vi "getSerializedData.vi"(0 "reference":refnum<class "NoteNode.lvclass">, 5 "error in (no error)":errorcluster) -> (14 "reference out":refnum<class "NoteNode.lvclass">, 15 "parent":refnum<class "AbstractNode.lvclass">, 16 "children":refnum<class "AbstractNode.lvclass">[](array[class]), 17 "xmlOut":string, 19 "error out":errorcluster)   [LabVIEW 2020, in "NoteNode.lvclass"]
doc: "getSerializedData"
uses:
  <resource>/Framework/Providers/Open_GDS/UML/NoteNode_class/NoteNode.lvclass
  C:/Program Files (x86)/National Instruments/LabVIEW 2020/resource/Framework/Providers/Open_GDS/UML/RectangularNode_class/RectangularNode.lvclass
  C:/Program Files (x86)/National Instruments/LabVIEW 2020/resource/Framework/Providers/Open_GDS/UML/AbstractNode_class/AbstractNode.lvclass
  <resource>/Framework/Providers/Open_GDS/UML/AbstractNode_class/AbstractNode.lvclass
  <resource>/Framework/Providers/Open_GDS/UML/General/Rectangle/Rectangle Rectangle2D.ctl
  <resource>/Framework/Providers/Open_GDS/UML/MultiLineString_class/JustificationType.ctl
  <resource>/Framework/Providers/Open_GDS/UML/MultiLineString_class/MultiLineString.lvclass
  <resource>/Framework/Providers/Open_GDS/UML/RectangularNode_class/RectangularNode.lvclass
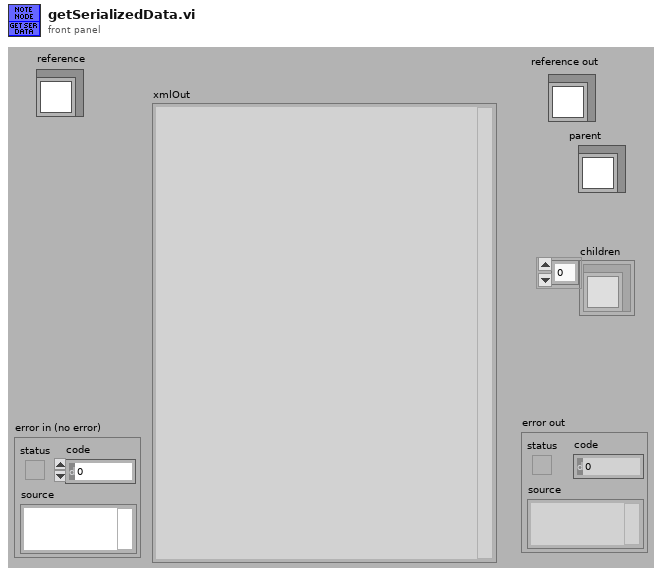
[diagram p1: front panel]
types:
  T1 = typedef "Rectangle Rectangle2D.ctl" = cluster{"x":dbl, "y":dbl, "width":dbl, "height":dbl}
  T2 = cluster{"Base class":cluster{"Base class":cluster{"parent":refnum<k1>, "children":refnum<k1>[], "Hidden":bool}, "bounds":T1}, "DEFAULT_WIDTH":i32, "DEFAULT_HEIGHT":i32, "DEFAULT_COLOR":u32, "FOLD_X":i32, "FOLD_Y":i32, "color":u32, "text":refnum<k1>, "pointNodes":refnum<k1>[]}
  T3 = typedef "MultiLineString.lvclass/JustificationType.ctl" = enum16{"LEFT", "CENTER", "RIGHT"}
  T4 = typedef "NoteNode.lvclass/ObjectAttributes.ctl" = cluster{"DEFAULT_WIDTH":i32, "DEFAULT_HEIGHT":i32, "DEFAULT_COLOR":u32, "FOLD_X":i32, "FOLD_Y":i32, "color":u32, "text":refnum<class "MultiLineString.lvclass">, "pointNodes":refnum<class "AbstractNode.lvclass">[]}
  T5 = typedef "RectangularNode.lvclass/ObjectAttributes.ctl" = cluster{"bounds":T1}
  T6 = typedef "AbstractNode.lvclass/ObjectAttributes.ctl" = cluster{"parent":refnum<class "AbstractNode.lvclass">, "children":refnum<class "AbstractNode.lvclass">[], "Hidden":bool}
  T7 = cluster{"Attributes":cluster{"Base class":cluster{"Base class":cluster{"parent":refnum<k1>, "children":refnum<k1>[], "Hidden":bool}, "bounds":T1}, "DEFAULT_WIDTH":i32, "DEFAULT_HEIGHT":i32, "DEFAULT_COLOR":u32, "FOLD_X":i32, "FOLD_Y":i32, "color":u32, "text":refnum<k1>, "pointNodes":refnum<k1>[]}, string}
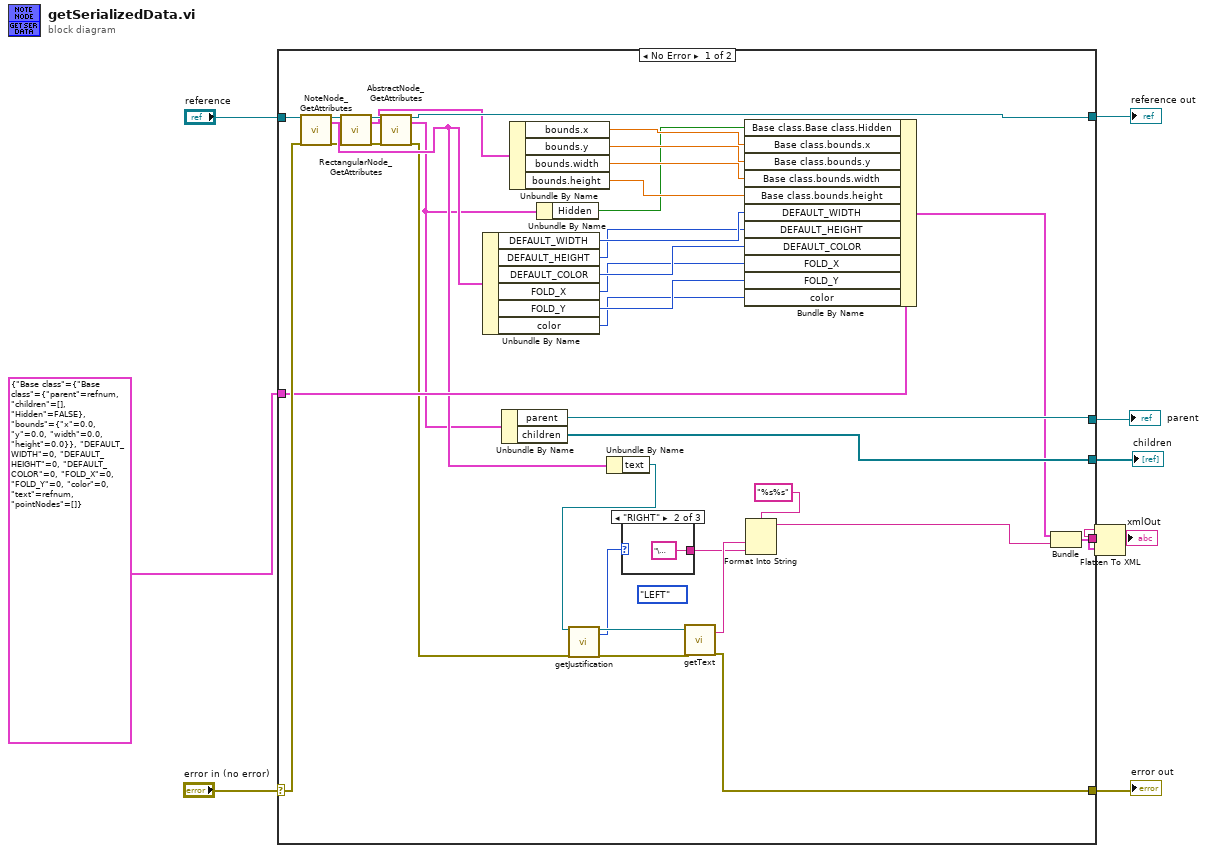
[diagram p0: block diagram]
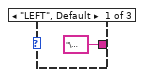
[diagram p2: hidden frame]
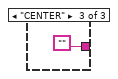
[diagram p3: hidden frame]
diagram:
  n1 = case shown="No Error" "error in (no error)" {
    selector: "error in (no error)" -> [w45 w49]
    tunnel: "reference" -> [w44 w50]
    tunnel: [w42 w49] -> w6
    tunnel: [w11 w50] -> w5
    tunnel: [w41 _] -> w4
    tunnel: [w40 _] -> w3
    tunnel: [w39 _] -> w2
    tunnel: T2 {"Base class"={"Base class"={"parent"=refnum, "children"=[], "Hidden"=FALSE}, "bounds"={"x"=0.0, "y"=0.0, "width"=0.0, "height"=0.0}}, "DEFAULT_WIDTH"=0, "DEFAULT_HEIGHT"=0, "DEFAULT_COLOR"=0, "FOLD_X"=0, "FOLD_Y"=0, "color"=0, "text"=refnum, "pointNodes"=[]} ("Attributes") -> [w30 _]
    frame No Error {
      (unwired) JustificationType."LEFT" ("justification")
      n2 = call <resource>:"NoteNode_GetAttributes.vi"("reference in"=w44, "error in (no error)"=w45) -> ("reference out"=w16:refnum<class "NoteNode.lvclass">, "Data"=w17:T4, "error out"=w15:errorcluster)  [unwired: 1 in, 14 out]
      n3 = call <resource>:"RectangularNode_GetAttributes.vi"("reference in"=w16, "error in (no error)"=w15) -> ("reference out"=w14:refnum<class "NoteNode.lvclass">, "Data"=w9:T5, "error out"=w13:errorcluster)  [unwired: 14 in, 1 out]
      n4 = call <resource>:"AbstractNode_GetAttributes.vi"("reference in"=w14, "error in (no error)"=w13) -> ("reference out"=w11:refnum<class "NoteNode.lvclass">, "Data"=w10:T6, "error out"=w12:errorcluster)  [unwired: 14 in, 1 out]
      n5 = Unbundle By Name(w17) -> ("DEFAULT_WIDTH"=w25:i32, "DEFAULT_HEIGHT"=w24:i32, "DEFAULT_COLOR"=w23:u32, "FOLD_X"=w22:i32, "FOLD_Y"=w21:i32, "color"=w20:u32)
      n6 = Unbundle By Name(w10) -> ("parent"=w41:refnum<class "AbstractNode.lvclass">, "children"=w40:refnum<class "AbstractNode.lvclass">[])
      n7 = Unbundle By Name(w9) -> ("bounds.x"=w29:dbl, "bounds.y"=w28:dbl, "bounds.width"=w27:dbl, "bounds.height"=w26:dbl)
      n8 = Unbundle By Name(w10) -> ("Hidden"=w18:bool)
      n9 = Unbundle By Name(w17) -> ("text"=w36:refnum<class "MultiLineString.lvclass">)
      n10 = call <resource>:"getJustification.vi"("reference"=w36, "error in (no error)"=w12) -> ("reference out"=w38:refnum<class "MultiLineString.lvclass">, "justification"=w32:T3, "error out"=w37:errorcluster)  [unwired: 15 out]
      n11 = case shown="\"RIGHT\"" w32 {
        tunnel: ["\u0001" "\u0003" ""] -> w31
        frame "LEFT", Default {
        }
        frame "RIGHT" {
        }
        frame "CENTER" {
        }
      }
      n12 = call-dynamic "getText.vi"("reference"=w38, "error in (no error)"=w37) -> ("text"=w34:string, "error out"=w42:errorcluster)  [unwired: 16 out]
      n13 = Bundle By Name(cluster=w30, "Base class.Base class.Hidden"=w18, "Base class.bounds.x"=w29, "Base class.bounds.y"=w28, "Base class.bounds.width"=w27, "Base class.bounds.height"=w26, "DEFAULT_WIDTH"=w25, "DEFAULT_HEIGHT"=w24, "DEFAULT_COLOR"=w23, "FOLD_X"=w22, "FOLD_Y"=w21, "color"=w20) -> (w19:T2)
      n14 = Format Into String(format string="%s%s", w34, w31) -> (resulting string=w33:string)  [unwired: 2 in, 1 out]
      n15 = Bundle("Attributes"=w19, w33) -> (w43:T7)  [unwired: 1 out]
      n16 = Flatten To XML(6:w43) -> (2:w39:string)
    }
    frame Error {
    }
  }
  "reference out" <- w5
  "error out" <- w6
  "parent" <- w4
  "children" <- w3
  "xmlOut" <- w2
